vi "Selection for Data folder.vi"(9 "Select":enum16{"Sample", "Blank"}(ring), 10 "F_array_Link":path[](array[path]), 11 "Folder_List":string[](array[string])) -> (2 "S_F_array_Link":path[](array[path]), 3 "S_Folder_List":string[](array[string]))   [LabVIEW 2018]
panel:
  out "Array":bool[](array[boolean])
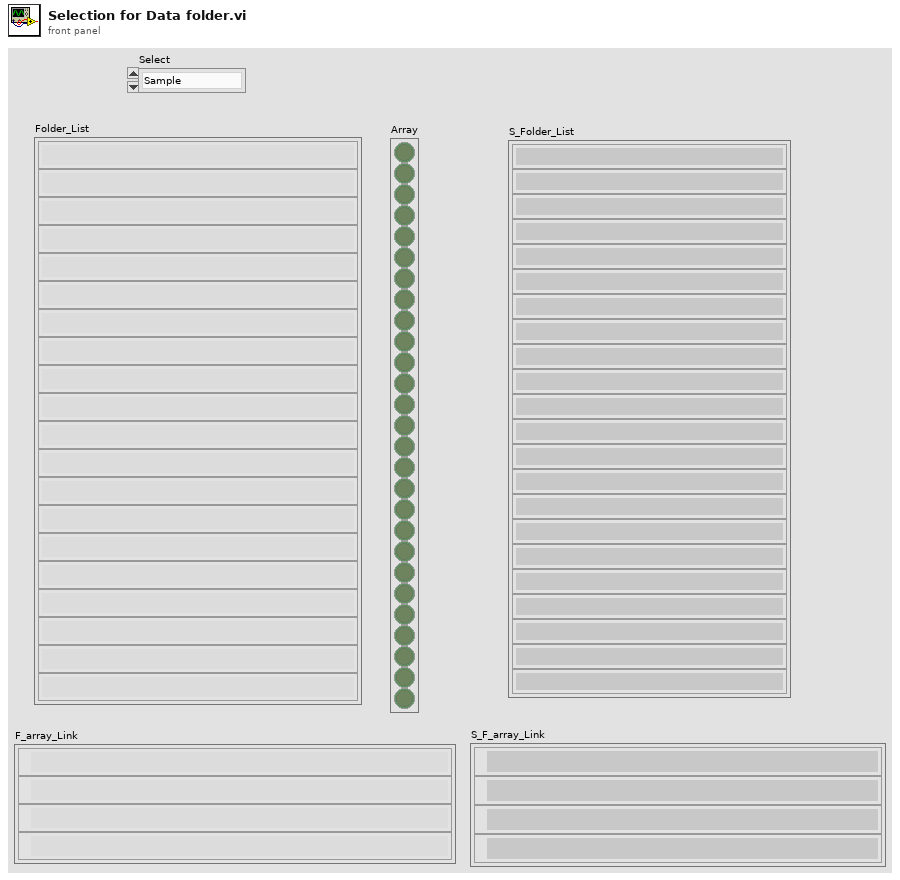
[diagram p1: front panel]
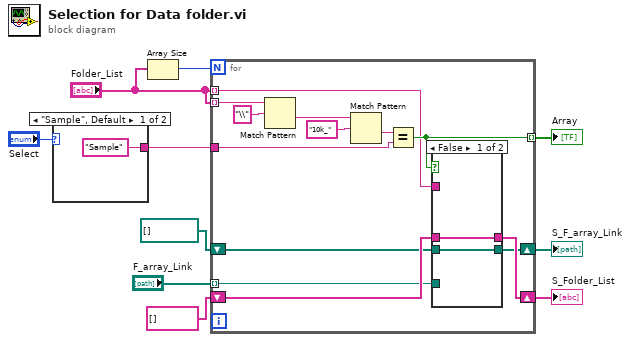
[diagram p0: block diagram]
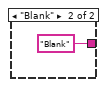
[diagram p2: hidden frame]
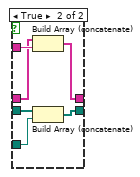
[diagram p3: hidden frame]
diagram:
  n1 = case shown="\"Sample\", Default" "Select" {
    tunnel: ["Sample" ("regular expression") "Blank" ("regular expression")] -> w1
    frame "Sample", Default {
    }
    frame "Blank" {
    }
  }
  n2 = Array Size(array="Folder_List") -> (size(s)=w10:i32)
  n3 = for {
    N: w10 -> [_]
    tunnel: "Folder_List" -> [w24] mode=indexing
    tunnel: [w20] -> w9 mode=indexing
    tunnel: "Folder_List" -> [w19] mode=indexing
    tunnel: "F_array_Link" -> [w16] mode=indexing
    shift-right: [w18] -> w5
    shift-left: string[] [] -> [w17]
    shift-right: [w15] -> w3
    shift-left: path[] [] -> [w14]
    tunnel: w1 -> [w13]
    n4 = Match Pattern(string=w24, regular expression="\\") -> (after substring=w22:string)  [unwired: 1 in, 3 out]
    n5 = Match Pattern(string=w22, regular expression="10k_") -> (after substring=w21:string)  [unwired: 1 in, 3 out]
    n6 = Equal?(x=w21, y=w13) -> (x = y?=w20:bool)
    n7 = case shown="False" w20 {
      tunnel: w19 -> [_ w33]
      tunnel: [w27 w32] -> w18
      tunnel: w17 -> [w27 w31]
      tunnel: w16 -> [_ w30]
      tunnel: [w26 w29] -> w15
      tunnel: w14 -> [w26 w28]
      frame False {
      }
      frame True {
        n8 = Build Array (concatenate)(w31, w33) -> (w32:string[])
        n9 = Build Array (concatenate)(w28, w30) -> (w29:path[])
      }
    }
  }
  "Array" <- w9
  "S_Folder_List" <- w5
  "S_F_array_Link" <- w3
